vi "Parse LTE Call Handover Param.vi"(8 "error in (no error)":errorcluster caption="에러 입력(에러 없음)", 10 "JSON string":string, 11 "Instrument Manager 입력":refnum<class "Instrument Manager.lvclass">) -> (0 "error out":errorcluster caption="에러 출력", 1 "LTE Call Handover Param":T1, 2 "Call Process Param LTE":T3, 3 "Instrument Manager 출력":refnum<class "Instrument Manager.lvclass">)   [LabVIEW 2023, in "Instrument Manager.lvclass"]
uses:
  Instrument Manager.lvclass
  Param Definition/Call Handover Param LTE.ctl
  Type Definition/LTE Call Handover Param.ctl
  Module/ANRITSU Call Box/Type Definition/LTE Supported BandWidth.ctl
  Instrument Manager.lvclass/Instrument Manager.ctl
  Module/ANRITSU Call Box/ANRITSU Call Box.lvlib
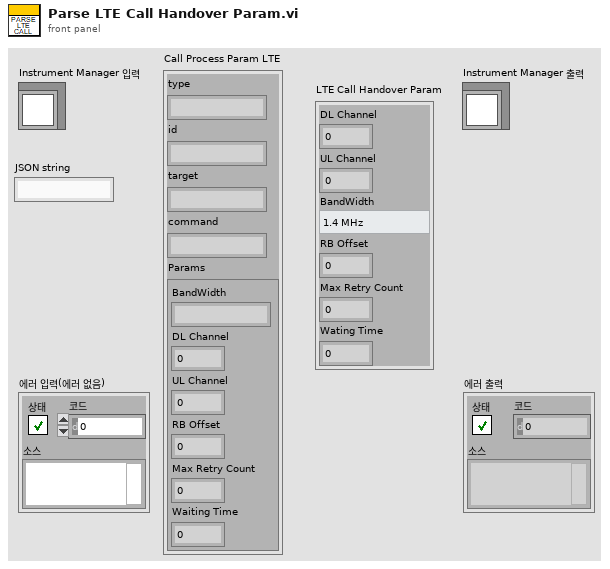
[diagram p1: front panel]
types:
  T1 = typedef "LTE Call Handover Param.ctl" = cluster{"DL Channel":i32, "UL Channel":i32, "BandWidth":T2, "RB Offset":i32, "Max Retry Count":i32, "Wating Time":i32}
  T2 = typedef "ANRITSU Call Box.lvlib/LTE Supported BandWidth.ctl" = enum16{"1.4 MHz", "3 MHz", "5 MHz", "10 MHz", "15 MHz", "20 MHz"}
  T3 = typedef "Instrument Manager.lvclass/Call Handover Param LTE.ctl" = cluster{"type":string, "id":string, "target":string, "command":string, "Params":cluster{"BandWidth":string, "DL Channel":i32, "UL Channel":i32, "RB Offset":i32, "Max Retry Count":i32, "Waiting Time":i32}}
  T4 = cluster{"BandWidth":string, "DL Channel":i32, "UL Channel":i32, "RB Offset":i32, "Max Retry Count":i32, "Waiting Time":i32}
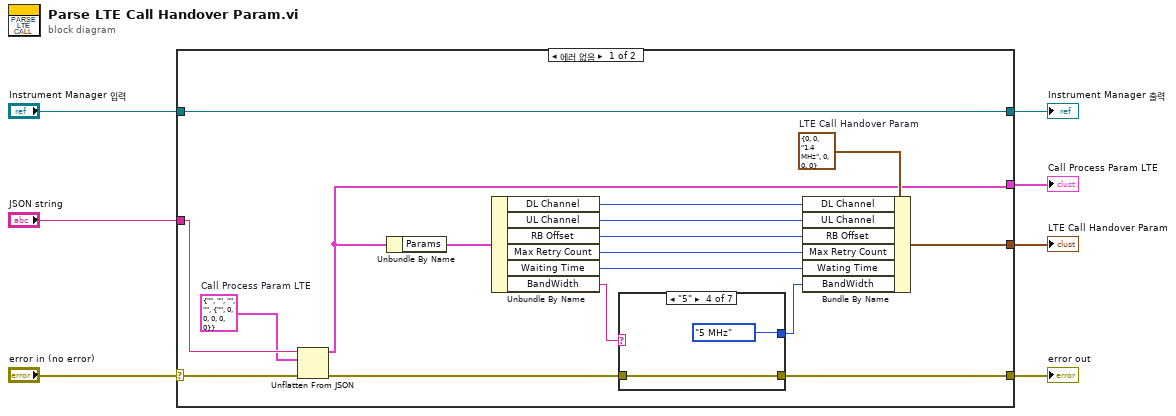
[diagram p0: block diagram]
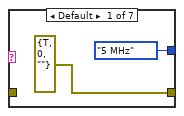
[diagram p2: hidden frame]
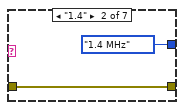
[diagram p3: hidden frame]
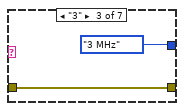
[diagram p4: hidden frame]
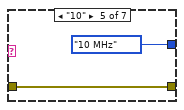
[diagram p5: hidden frame]
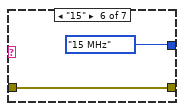
[diagram p6: hidden frame]
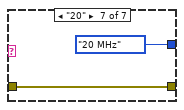
[diagram p7: hidden frame]
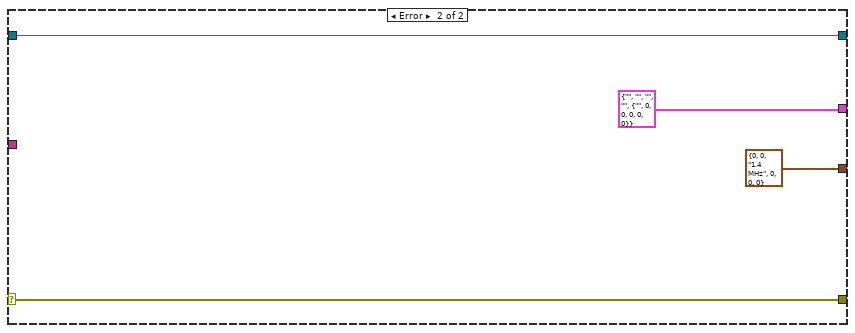
[diagram p8: hidden frame]
diagram:
  n1 = case shown="에러 없음" "error in (no error)" {
    selector: "error in (no error)" -> [w23 w42]
    tunnel: [w13 w42] -> w3
    tunnel: [w24 w41] -> w4
    tunnel: "Instrument Manager 입력" -> [w24 w41]
    tunnel: "JSON string" -> [w22 _]
    tunnel: [w9 T1 {"DL Channel"=0, "UL Channel"=0, "BandWidth"=enum."1.4 MHz", "RB Offset"=0, "Max Retry Count"=0, "Wating Time"=0} ("LTE Call Handover Param")] -> w2
    tunnel: [w8 T3 {"type"="", "id"="", "target"="", "command"="", "Params"={"BandWidth"="", "DL Channel"=0, "UL Channel"=0, "RB Offset"=0, "Max Retry Count"=0, "Waiting Time"=0}} ("Call Process Param LTE")] -> w1
    frame No Error {
      w10 = T3 {"type"="", "id"="", "target"="", "command"="", "Params"={"BandWidth"="", "DL Channel"=0, "UL Channel"=0, "RB Offset"=0, "Max Retry Count"=0, "Waiting Time"=0}}  # Call Process Param LTE
      w11 = T1 {"DL Channel"=0, "UL Channel"=0, "BandWidth"=enum."1.4 MHz", "RB Offset"=0, "Max Retry Count"=0, "Wating Time"=0}  # LTE Call Handover Param
      n2 = Unflatten From JSON(JSON string=w22, type and defaults=w10, error in (no error)=w23) -> (value=w8:T3, error out=w14:errorcluster)  [unwired: 4 in]
      n3 = Unbundle By Name(w8) -> ("Params"=w15:T4)
      n4 = Unbundle By Name(w15) -> ("DL Channel"=w12:i32, "UL Channel"=w19:i32, "RB Offset"=w18:i32, "Max Retry Count"=w17:i32, "Waiting Time"=w16:i32, "BandWidth"=w21:string)
      n5 = case shown="\"5\"" w21 {
        tunnel: w14 -> [_ w28 w30 w32 w33 w35 w37]
        tunnel: [errorcluster {"status"=TRUE, "code"=0, "source"=""} ("error out") w28 w30 w32 w33 w35 w37] -> w13
        tunnel: [LTE_Supported_BandWidth."5 MHz" ("BandWidth") LTE_Supported_BandWidth."1.4 MHz" ("BandWidth") LTE_Supported_BandWidth."3 MHz" ("BandWidth") LTE_Supported_BandWidth."5 MHz" ("BandWidth") LTE_Supported_BandWidth."10 MHz" ("BandWidth") LTE_Supported_BandWidth."15 MHz" ("BandWidth") LTE_Supported_BandWidth."20 MHz" ("BandWidth")] -> w20
        frame Default {
        }
        frame "1.4" {
        }
        frame "3" {
        }
        frame "5" {
        }
        frame "10" {
        }
        frame "15" {
        }
        frame "20" {
        }
      }
      n6 = Bundle By Name(cluster=w11, "DL Channel"=w12, "UL Channel"=w19, "RB Offset"=w18, "Max Retry Count"=w17, "Wating Time"=w16, "BandWidth"=w20) -> (w9:T1)
    }
    frame Error {
    }
  }
  "error out" <- w3
  "Instrument Manager 출력" <- w4
  "Call Process Param LTE" <- w1
  "LTE Call Handover Param" <- w2
